vi "D_Check_FMem_Slot.vi"(6 "YPixel":u32, 7 "XPixel":u32, 8 "error in (no error)":errorcluster, 10 "slotNo":u32, 11 "bID":u8) -> (0 "error out":errorcluster, 2 "Read array":u8[][](array[numeric]), 3 "bID":u8, 4 "TorF":i32)   [LabVIEW 2018]
uses:
  hpkSLMdaLV.dll
panel:
  out "Read image":picture
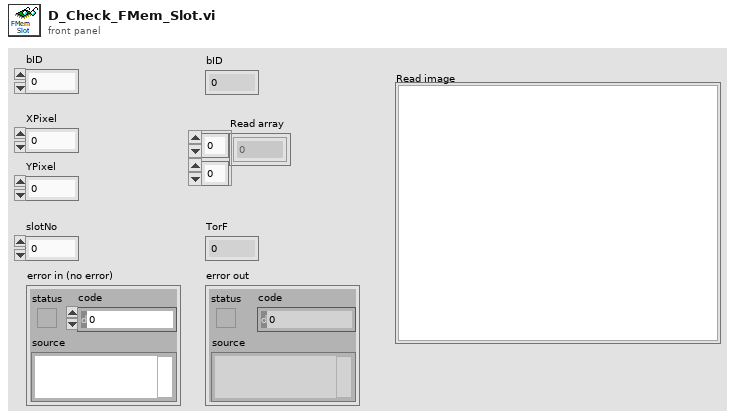
[diagram p1: front panel]
types:
  T1 = typedef "imagedata.ctl" = cluster{"image type":i32, "image depth":i32, "image":u8[], "mask":u8[], "colors":u32[], "Rectangle":cluster{"left":i16, "top":i16, "right":i16, "bottom":i16}}
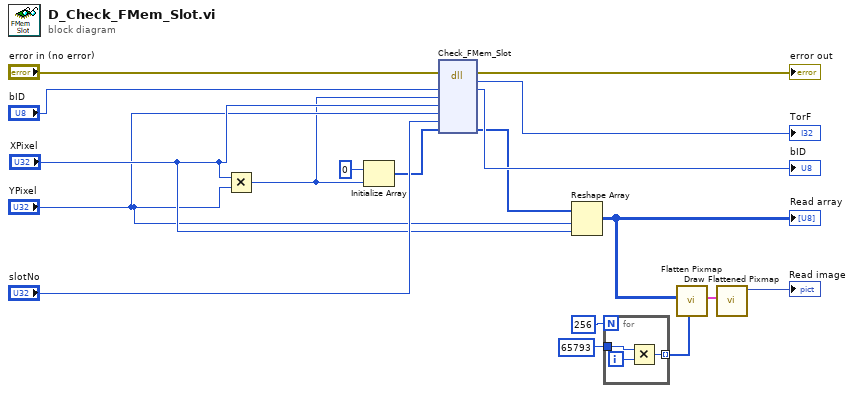
[diagram p0: block diagram]
diagram:
  n1 = Multiply(x="XPixel", y="YPixel") -> (x*y=w9:u32)
  n2 = Initialize Array(u8 0, w9) -> (w8:u8[])
  n3 = dll-call lib="PTH2ﾅunc \\\\K45292-FS\\Data\n荳ｭ遐猫COSpost譛晉ｨｲ\n08_LabVIEW!00_繝ｩ繝懊ン繝･繝ｼ繝励Ο繧ｰ繝ｩ繝LabVIEW2018 LCOS_DriverV3.0_Hardware_ControlUSB_Multi-ControlHardwareControl_LVhpkSLMdaLV.dll" fn="Check_FMem_Slot"(error in="error in (no error)", "bID"="bID", "arraySize"=w9, "XPixel"="XPixel", "YPixel"="YPixel", "slotNo"="slotNo", "readArray"=w8) -> (error out=→"error out":errorcluster, "返り値タイプ"=→"TorF":i32, "bID"=→"bID":u8, "readArray"=w7:u8[])  [unwired: 6 in, 1 out]
  n4 = Reshape Array(w7, "YPixel", "XPixel") -> (w2:u8[][])
  "Read array" <- w2
  n5 = for {
    N: 256 -> [_]
    tunnel: 65793 -> [w20]
    tunnel: [w19] -> w6 mode=indexing
    i -> [w21]
    n6 = Multiply(x=w20, y=w21) -> (x*y=w19:i32)
  }
  n7 = call <vilib>:"Flatten Pixmap.vi"("colors"=w6, "8-bit pixmap"=w2) -> ("image data"=w5:T1)  [unwired: 9 in]
  n8 = call <vilib>:"Draw Flattened Pixmap.vi"("image data"=w5) -> ("new picture"=→"Read image":picture)  [unwired: 8 in]
